vi "MaP test_fonction.vi"() -> ()   [LabVIEW 2020]
uses:
  LabVIEW-Python TCP Lib/LabVIEW-Python TCP Lib.lvlib
panel:
  in  "Lancer server.py":string=" \"D:\\Home\\eschaub\\Documents\\INFORMATIQUE\\LabVIEW-Python TCP\\lancer_serveur.py\""
  out "Stop server message":string
  out "value":cluster{"nom":string, "Numeric":dbl}[](array[cluster])
  out "data string out":string
  in  "Cluster_de_depart":cluster{"fonction":string}={"fonction"="test_fonction"}
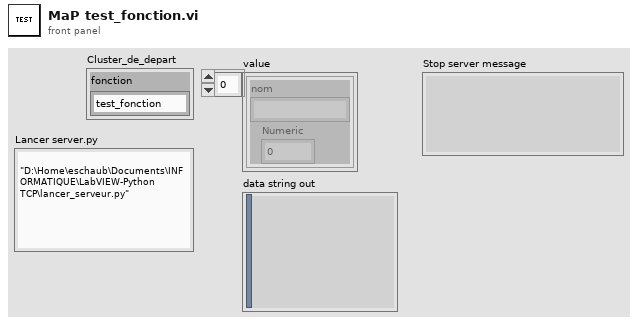
[diagram p1: front panel]
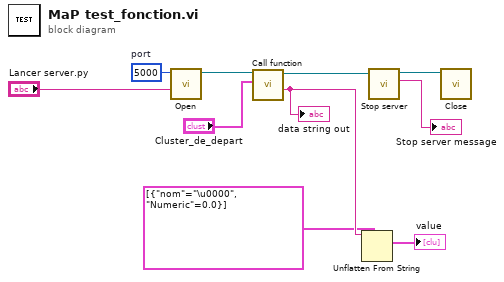
[diagram p0: block diagram]
diagram:
  w5 = u16 5000  # port
  n1 = call "Open.vi"("Lancer server.py"="Lancer server.py", "port"=w5) -> ("connection ID"=w10:refnum<k5>)  [unwired: 8 in, 1 out]
  n2 = call "Call function.vi"("variant in"="Cluster_de_depart", "connection ID"=w10) -> ("data string out"=w8:string, "connection ID out"=w4:refnum<k5>)  [unwired: 6 in, 2 out]
  "data string out" <- w8
  n3 = Unflatten From String(type=cluster{"nom":string, "Numeric":dbl}[] [{"nom"="\u0000", "Numeric"=0.0}], binary string=w8) -> (value=→"value":cluster{"nom":string, "Numeric":dbl}[])  [unwired: 3 in, 2 out]
  n4 = call "Stop server.vi"("connection ID"=w4) -> ("Stop server message"=→"Stop server message":string, "connection ID out"=w3:refnum<k5>)  [unwired: 8 in, 1 out]
  n5 = call "Close.vi"("connection ID"=w3) -> ()  [unwired: 9 in, 2 out]
